vi "PlcToPCArrayTrans(SubVI).vi"(8 "error in (no error)":errorcluster caption="에러 입력(에러 없음)", 11 "PLC배열입력":u16[][](array[numeric])) -> (0 "error out":errorcluster caption="에러 출력", 3 "PLCArrayToTrans":u16[](array[numeric]))   [LabVIEW 2019]
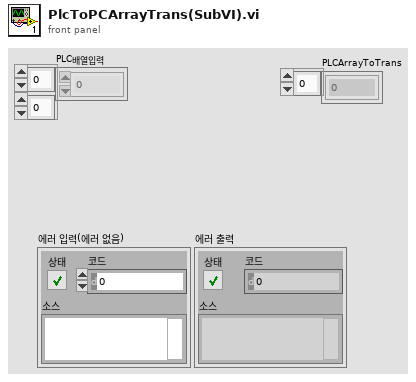
[diagram p1: front panel]
types:
  T1 = cluster{"PLC배열입력[0]":u16, "PLC배열입력[1]":u16, "PLC배열입력[2]":u16, "PLC배열입력[3]":u16, "PLC배열입력[4]":u16, "PLC배열입력[5]":u16, "PLC배열입력[6]":u16, "PLC배열입력[7]":u16, "PLC배열입력[8]":u16}
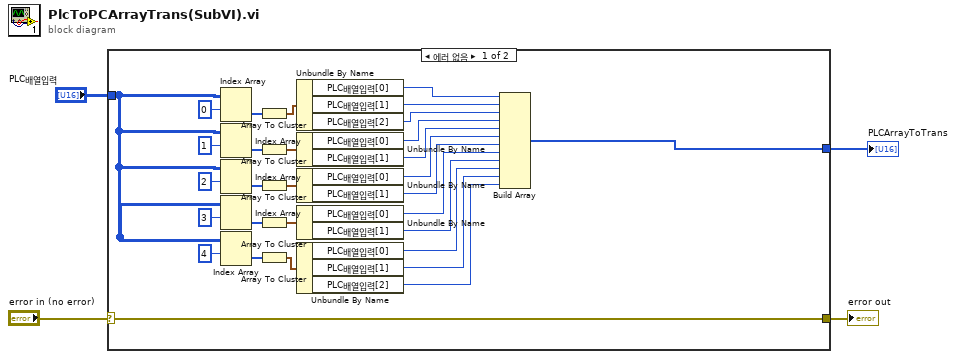
[diagram p0: block diagram]
diagram:
  n1 = case shown="에러 없음" "error in (no error)" {
    selector: "error in (no error)" -> [w19 w35]
    tunnel: [w19 w35] -> w3
    tunnel: "PLC배열입력" -> [w18 _]
    tunnel: [w11 _] -> w1
    frame No Error {
      n2 = Index Array(array=w18, index (row)=0 ("인덱스 (행)")) -> (element=w25:u16[])  [unwired: 1 in]
      n3 = Index Array(array=w18, index (row)=1 ("인덱스 (행)")) -> (element=w26:u16[])  [unwired: 1 in]
      n4 = Index Array(array=w18, index (row)=2 ("인덱스 (행)")) -> (element=w29:u16[])  [unwired: 1 in]
      n5 = Index Array(array=w18, index (row)=3 ("인덱스 (행)")) -> (element=w28:u16[])  [unwired: 1 in]
      n6 = Index Array(array=w18, index (row)=4 ("인덱스 (행)")) -> (element=w27:u16[])  [unwired: 1 in]
      n7 = Array To Cluster(array=w25) -> (cluster=w30:T1)
      n8 = Array To Cluster(array=w26) -> (cluster=w31:T1)
      n9 = Array To Cluster(array=w29) -> (cluster=w32:T1)
      n10 = Array To Cluster(array=w28) -> (cluster=w33:T1)
      n11 = Array To Cluster(array=w27) -> (cluster=w34:T1)
      n12 = Unbundle By Name(w30) -> ("PLC배열입력[0]"=w10:u16, "PLC배열입력[1]"=w9:u16, "PLC배열입력[2]"=w8:u16)
      n13 = Unbundle By Name(w31) -> ("PLC배열입력[0]"=w17:u16, "PLC배열입력[1]"=w16:u16)
      n14 = Unbundle By Name(w32) -> ("PLC배열입력[0]"=w15:u16, "PLC배열입력[1]"=w14:u16)
      n15 = Unbundle By Name(w33) -> ("PLC배열입력[0]"=w13:u16, "PLC배열입력[1]"=w12:u16)
      n16 = Unbundle By Name(w34) -> ("PLC배열입력[0]"=w7:u16, "PLC배열입력[1]"=w6:u16, "PLC배열입력[2]"=w5:u16)
      n17 = Build Array(w10, w9, w8, w17, w16, w15, w14, w13, w12, w7, w6, w5) -> (w11:u16[])
    }
    frame Error {
    }
  }
  "error out" <- w3
  "PLCArrayToTrans" <- w1
